vi "ClimbOutput.vi"(10 "Driver Right Bumper":bool, 11 "Driver Left Bumper":bool) -> (2 "Rear Climb Output":T1, 3 "Front Climb Output":T1)   [LabVIEW 2018]
uses:
  <vilib>/Rock Robotics/WPI/Solenoid/WPI_SolenoidValue.ctl
  Robot Global Data.vi
panel:
  out "ClimbOutput":dbl
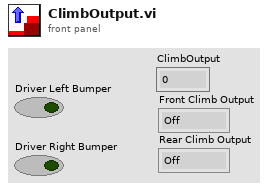
[diagram p1: front panel]
types:
  T1 = typedef "WPI_SolenoidValue.ctl" = enum16{"Off", "On", "Forward", "Reverse"}
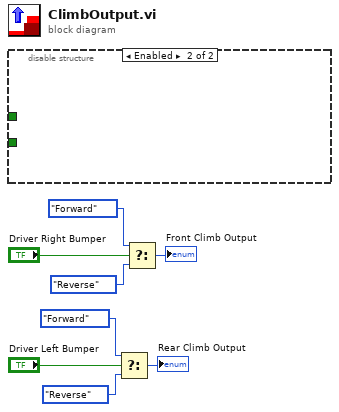
[diagram p0: block diagram]
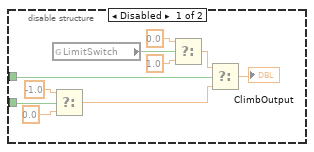
[diagram p2: hidden frame]
diagram:
  n1 = disable-structure shown="Enabled" {
    disable-tunnel: _ -> [w16 _]
    disable-tunnel: _ -> [w9 _]
    frame Disabled {
      n2 = global read "Robot Global Data.vi" "LimitSwitch"() -> (w10:bool)
      n3 = Select(t=-1.0, s=w16, f=0.0) -> (s? t:f=w18:dbl)
      n4 = Select(t=0.0, s=w10, f=1.0 ("t")) -> (s? t:f=w12:dbl)
      n5 = Select(t=w12, s=w9, f=w18) -> (s? t:f=→"ClimbOutput":dbl)
    }
    frame Enabled {
    }
  }
  n6 = Select(t=WPI_SolenoidValue."Forward" ("Value"), s="Driver Left Bumper", f=WPI_SolenoidValue."Reverse" ("Value")) -> (s? t:f=→"Rear Climb Output":T1)
  n7 = Select(t=WPI_SolenoidValue."Forward" ("Value"), s="Driver Right Bumper", f=WPI_SolenoidValue."Reverse" ("Value")) -> (s? t:f=→"Front Climb Output":T1)
